vi "Ecrire config EDWARDS grappes.vi"(8 "entrée d'erreur (pas d'erreur)":errorcluster, 10 "Grappes":string[][](array[string]), 11 "Refnum en entrée":T1 caption="refnum out") -> (0 "sortie d'erreur":errorcluster, 1 "Sélect Grappes":bool[](array[boolean]), 2 "Seuil Jauge":T2={"Descente en Pression"={"Min Mesure Piezo"=5.0, "Min Mesure Pirani"=0.0002}, "Montée en Pression"={"Max Mesure Pirani"=10.0, "Max Mesure Penning"=0.0004}} {"Montée en Pression"."Max Mesure Penning" format="%.2e"; "Montée en Pression"."Max Mesure Pirani" format="%.2e"; "Descente en Pression"."Min Mesure Pirani" format="%.2e"; "Descente en Pression"."Min Mesure Piezo" format="%.2e"}, 3 "Refnum en sortie":T1 caption="refnum out")   [LabVIEW 2022 SP3]
uses:
  Gestion grappe/TypeDef_Seuil Jauge Pression_CN.ctl
  <vilib>/Utility/config.llb/Config Data RefNum.ctl
  Variables globales/Variable glob Edwards.vi
  <vilib>/Utility/config.llb/Write Key (String).vi
  <vilib>/Utility/config.llb/Write Key (Boolean).vi
  <vilib>/Utility/config.llb/Write Key (Double).vi
  <vilib>/Utility/config.llb/NI_LVConfig.lvlib
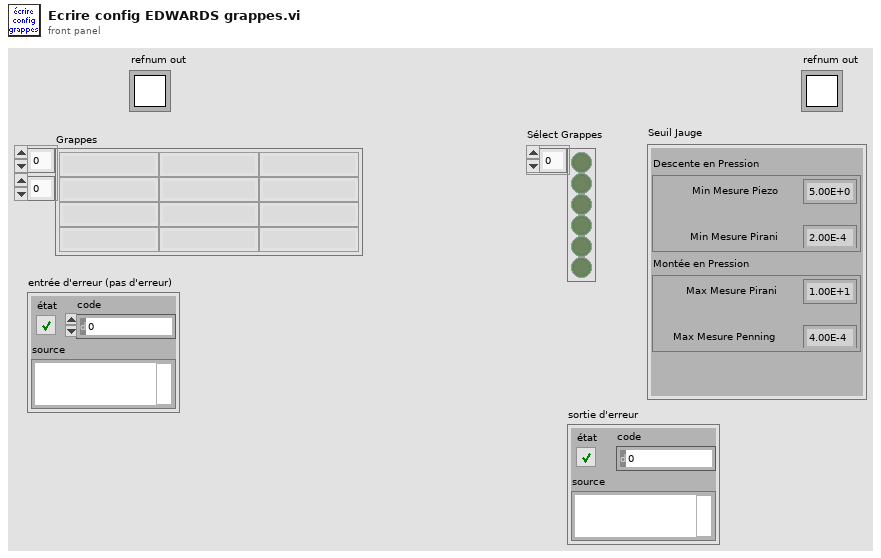
[diagram p1: front panel]
types:
  T1 = typedef "NI_LVConfig.lvlib/Config Data RefNum.ctl" = refnum<k1>
  T2 = typedef "TypeDef_Seuil Jauge Pression_CN.ctl" = cluster{"Descente en Pression":cluster{"Min Mesure Piezo":dbl, "Min Mesure Pirani":dbl}, "Montée en Pression":cluster{"Max Mesure Pirani":dbl, "Max Mesure Penning":dbl}}
  T3 = enum16{"fractional", "engineering", "exponential"}
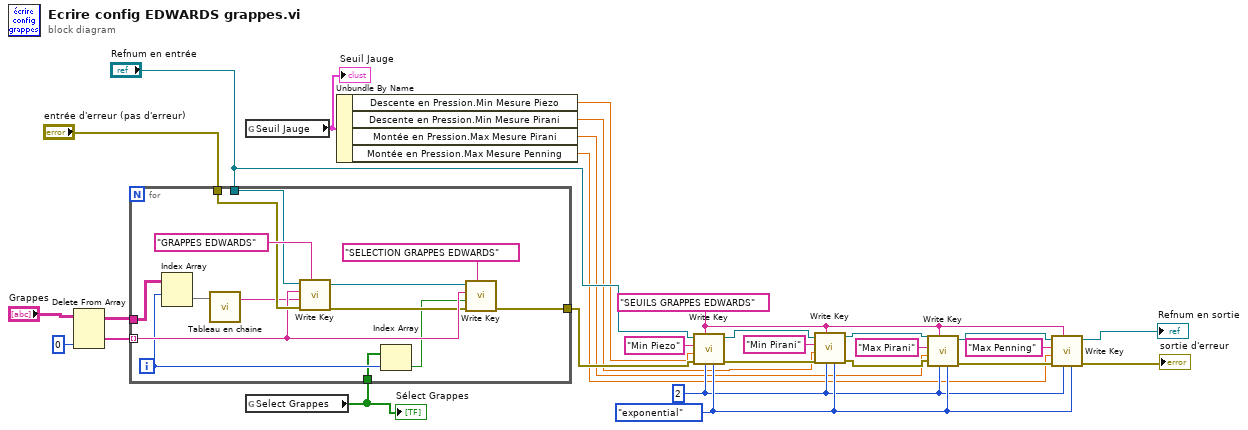
[diagram p0: block diagram]
diagram:
  w25 = i16 2 ("precision (6)")
  w26 = T3."exponential" ("format (fractional)")
  w14 = "SEUILS GRAPPES EDWARDS" ("section")
  n1 = Delete From Array(array="Grappes", index (col)=0 ("indice désactivé (col)")) -> (deleted portion=w3:string[], array with subset deleted=w5:string[][])  [unwired: 2 in]
  n2 = global read "Variable glob Edwards.vi" "Seuil Jauge"() -> (w24:T2)
  "Seuil Jauge" <- w24
  n3 = global read "Variable glob Edwards.vi" "Select Grappes"() -> (w6:bool[])
  "Sélect Grappes" <- w6
  n4 = for {
    tunnel: w3 -> [w38] mode=indexing
    tunnel: w5 -> [w34]
    tunnel: [w35] -> w27
    tunnel: "Refnum en entrée" -> [w41]
    tunnel: "entrée d'erreur (pas d'erreur)" -> [w40]
    tunnel: w6 -> [w32]
    i -> [w33]
    n5 = Index Array(array=w34, index (row)=w33) -> (element=w30:string[])  [unwired: 1 in]
    n6 = call "Tableau en chaine.vi"("Tableau 1D"=w30) -> ("Chaîne"=w29:string)  [unwired: 1 in, 1 out]
    n7 = call-poly <vilib>:"Write Key.vi"("section"="GRAPPES EDWARDS", "error in (no error)"=w40, "value"=w29, "key"=w38, "refnum"=w41) -> ("error out"=w36:errorcluster, "refnum out"=w37:T1)  [unwired: 4 in, 1 out]
    n8 = Index Array(array=w32, index=w33) -> (element=w31:bool)
    n9 = call-poly <vilib>:"Write Key.vi"("section"="SELECTION GRAPPES EDWARDS", "error in (no error)"=w36, "value"=w31, "key"=w38, "refnum"=w37) -> ("error out"=w35:errorcluster)  [unwired: 4 in, 2 out]
  }
  n10 = Unbundle By Name(w24) -> ("Descente en Pression.Min Mesure Piezo"=w9:dbl, "Descente en Pression.Min Mesure Pirani"=w10:dbl, "Montée en Pression.Max Mesure Pirani"=w12:dbl, "Montée en Pression.Max Mesure Penning"=w15:dbl)
  n11 = call-poly <vilib>:"Write Key.vi"("format (fractional)"=w26, "precision (6)"=w25, "section"=w14, "error in (no error)"=w27, "value"=w9, "key"="Min Piezo", "refnum"="Refnum en entrée") -> ("error out"=w16:errorcluster, "refnum out"=w19:T1)  [unwired: 2 in, 1 out]
  n12 = call-poly <vilib>:"Write Key.vi"("format (fractional)"=w26, "precision (6)"=w25, "section"=w14, "error in (no error)"=w16, "value"=w10, "key"="Min Pirani", "refnum"=w19) -> ("error out"=w17:errorcluster, "refnum out"=w20:T1)  [unwired: 2 in, 1 out]
  n13 = call-poly <vilib>:"Write Key.vi"("format (fractional)"=w26, "precision (6)"=w25, "section"=w14, "error in (no error)"=w17, "value"=w12, "key"="Max Pirani", "refnum"=w20) -> ("error out"=w18:errorcluster, "refnum out"=w21:T1)  [unwired: 2 in, 1 out]
  n14 = call-poly <vilib>:"Write Key.vi"("format (fractional)"=w26, "precision (6)"=w25, "section"=w14, "error in (no error)"=w18, "value"=w15, "key"="Max Penning", "refnum"=w21) -> ("error out"=→"sortie d'erreur":errorcluster, "refnum out"=→"Refnum en sortie":T1)  [unwired: 2 in, 1 out]
